vi "DepthProfileWriteCore.vi"(7 "Buffer In":T1(array[cluster]), 8 "error in":errorcluster, 9 "RepRate (Hz)":dbl=500.0, 10 "Total_Depth (shots)":i32=500, 11 "pre-Processed_Buffer":refnum<queue>) -> (0 "error out":errorcluster, 5 "Buffer Out":T1(array[cluster]))   [LabVIEW 2013]
panel:
  out "Array":i32[](array[numeric])
  out "# elements in queue":i32
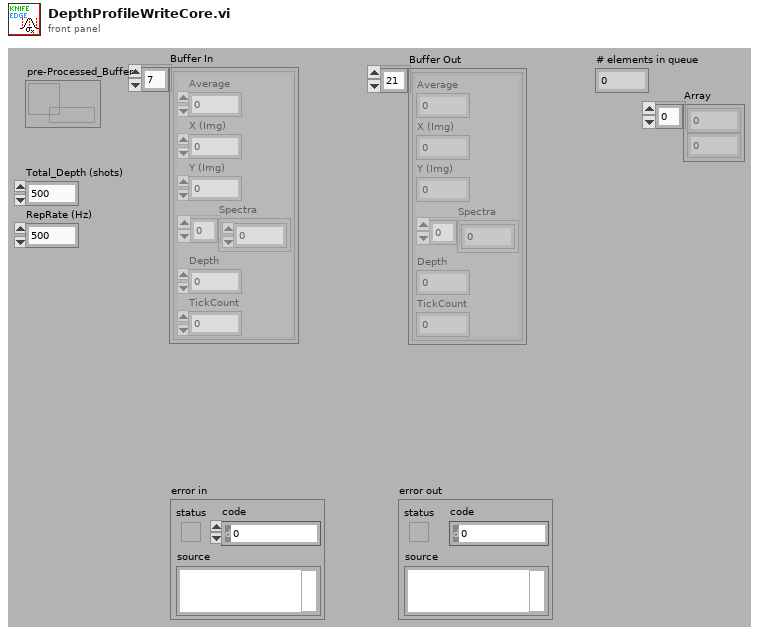
[diagram p1: front panel]
types:
  T1 = cluster{"Average":i32, "X (Img)":i32, "Y (Img)":i32, "Spectra":sgl[], "Depth":i32, "TickCount":dbl}[]
  T2 = cluster{"Average":i32, "X (Img)":i32, "Y (Img)":i32, "Spectra":sgl[], "Depth":i32, "TickCount":dbl}
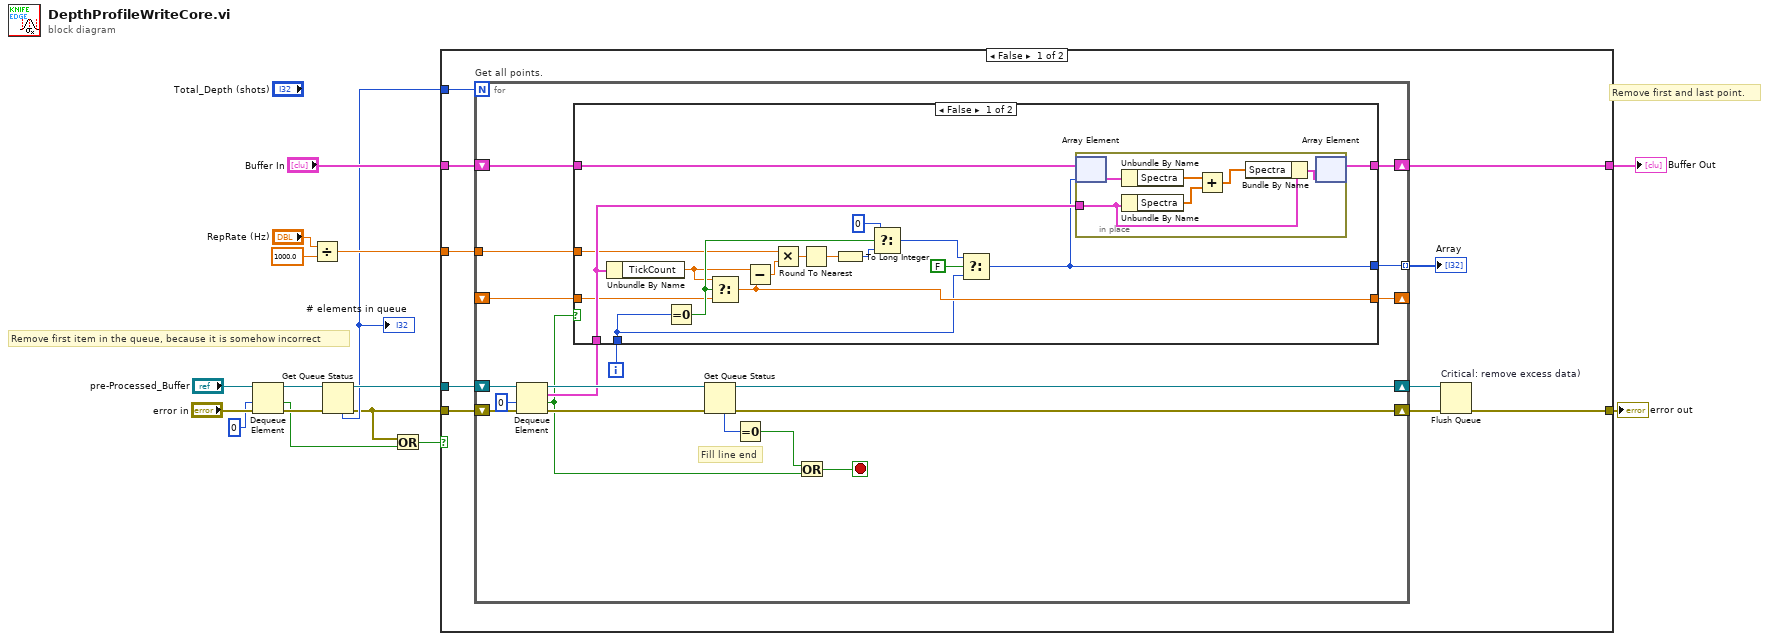
[diagram p0: block diagram]
diagram:
  # "Remove first item in the queue, because it is somehow incorrect"
  # "Remove first and last point."
  n1 = Dequeue Element ("Somehow, the first item is empty not real signal.")(queue="pre-Processed_Buffer", timeout in ms (-1)=0, error in (no error)="error in") -> (queue out=w12:refnum<queue>, timed out?=w1:bool, error out=w6:errorcluster)  [unwired: 1 out]
  n2 = Divide(x="RepRate (Hz)", y=1000.0 ("x")) -> (x/y=w14:dbl)
  n3 = Get Queue Status(queue=w12, error in (no error)=w6) -> (queue out=w7:refnum<queue>, error out=w2:errorcluster, # elements in queue=w5:i32)  [unwired: 1 in, 5 out]
  "# elements in queue" <- w5
  n4 = Or(x=w2, y=w1) -> (x .or. y?=w3:bool)
  n5 = case shown="False" w3 {
    tunnel: [w22 w70] -> w16
    tunnel: w7 -> [w19 _]
    tunnel: w5 -> [w26 _]
    tunnel: w14 -> [w25 _]
    tunnel: "Buffer In" -> [w21 w71]
    tunnel: [w20 w71] -> w8
    tunnel: w2 -> [w18 w70]
    frame False {
      n6 = for "Get all points." {
        N: w26 -> [_]
        shift-right: [w42] -> w24
        shift-left: w18 -> [w44]
        shift-right: [w38] -> w20
        shift-left: w21 -> [w39]
        shift-right: [w32] -> _
        shift-left: _ -> [w34]
        tunnel: w25 -> [w33]
        shift-right: [w31] -> w23
        shift-left: w19 -> [w43]
        tunnel: [w27] -> w17 mode=indexing
        i -> [w35]
        stop <- w29 stop-if-true
        # "Fill line end"
        n7 = Dequeue Element(queue=w43, timeout in ms (-1)=0, error in (no error)=w44) -> (queue out=w41:refnum<queue>, element=w36:T2, timed out?=w28:bool, error out=w42:errorcluster)
        n8 = case shown="False" w28 {
          tunnel: w39 -> [w61 w69]
          tunnel: [w60 w69] -> w38
          tunnel: w36 -> [w59 _]
          tunnel: w35 -> [w47 _]
          tunnel: w34 -> [w56 w68]
          tunnel: w33 -> [w53 _]
          tunnel: [w51 w68] -> w32
          tunnel: [w46 _] -> w27
          frame False {
            n9 = Unbundle By Name(w59) -> ("TickCount"=w55:dbl)
            n10 = Equal To 0?(x=w47) -> (x = 0?=w58:bool)
            n11 = Select(t=w55, s=w58, f=w56) -> (s? t:f=w51:dbl)
            n12 = Subtract(x=w55, y=w51) -> (x-y=w50:dbl)
            n13 = Multiply(x=w53, y=w50) -> (x*y=w54:dbl)
            n14 = Round To Nearest(number=w54) -> (nearest integer value=w52:dbl)
            n15 = To Long Integer(number=w52) -> (32bit integer=w49:i32)
            n16 = Select(t=0, s=w58, f=w49) -> (s? t:f=w45:i32)
            n17 = Select(t=w45, s=FALSE, f=w47) -> (s? t:f=w46:i32)
            n18 = in-place {
              in-place-border: w59 -> [w63]
              n19 = in-place-array #1(w61, w46) -> (w67:T2)
              n20 = Unbundle By Name(w67) -> ("Spectra"=w66:sgl[])
              n21 = Unbundle By Name(w63) -> ("Spectra"=w65:sgl[])
              n22 = Add(x=w66, y=w65) -> (x+y=w62:sgl[])
              n23 = Bundle By Name(cluster=w63, "Spectra"=w62) -> (w64:T2)
              n24 = in-place-array #1(w64) -> (w60:T1)  [unwired: 1 out]
            }
          }
          frame True {
          }
        }
        n25 = Get Queue Status(queue=w41) -> (queue out=w31:refnum<queue>, # elements in queue=w40:i32)  [unwired: 2 in, 6 out]
        n26 = Equal To 0?(x=w40) -> (x = 0?=w37:bool)
        n27 = Or(x=w37, y=w28) -> (x .or. y?=w29:bool)
      }
      "Array" <- w17
      n28 = Flush Queue "Critical: remove excess data)"(queue=w23, error in (no error)=w24) -> (error out=w22:errorcluster)  [unwired: 2 out]
    }
    frame True {
    }
  }
  "error out" <- w16
  "Buffer Out" <- w8
